vi "Bridge_Acquire_Lease.vi"(8 "error in (no error)":errorcluster={"status"=FALSE, "code"=0, "source"="\"\""}, 10 "run/step owner":string, 11 "Resource IDs":string) -> (0 "error out":errorcluster={"status"=FALSE, "code"=0, "source"="\"\""}, 2 "status ok":bool, 3 "Lease token / busy status":string)   [LabVIEW 2026]
doc: "INTENT: Grant exclusive write control. LOGIC: Atomically verify requested set then allocate bounded leases and expiry policy."
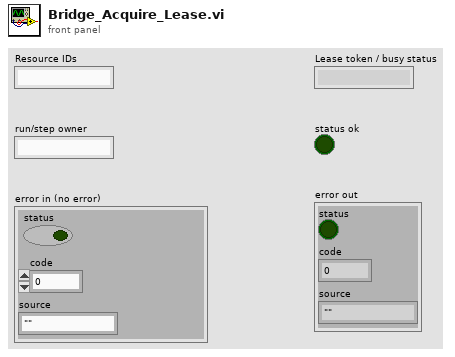
[diagram p1: front panel]
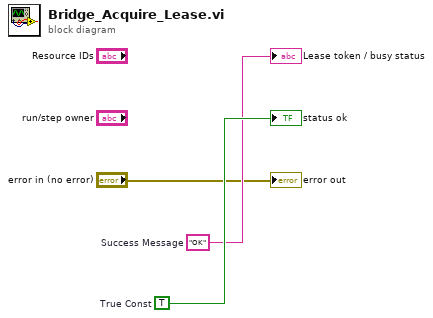
[diagram p0: block diagram]
diagram:
  w3 = TRUE  # True Const
  w2 = "OK"  # Success Message
  "Lease token / busy status" <- w2
  "status ok" <- w3
  "error out" <- "error in (no error)"
